vi "Close Item Reference.vi"(8 "error in (no error)":errorcluster, 11 "VI in":refnum<class "VI.lvclass">) -> (0 "error out":errorcluster, 3 "VI out":refnum<class "VI.lvclass">)   [LabVIEW 2020, in "VI Properties Editor.lvlib" / "VI.lvclass"]
doc: "Closes the reference contained within the class data of <B>VI in</B>."
uses:
  VI.lvclass
  VI.lvclass/VI.ctl
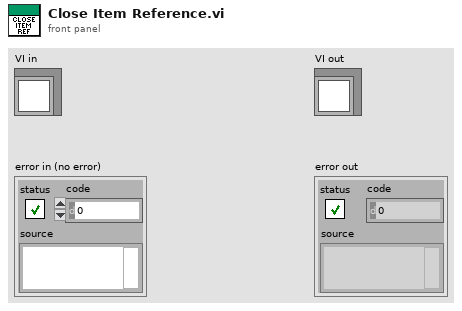
[diagram p1: front panel]
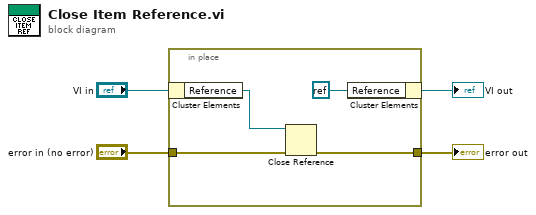
[diagram p0: block diagram]
diagram:
  n1 = in-place {
    in-place-border: "error in (no error)" -> [w8]
    in-place-border: [w5] -> w1
    n2 = in-place-cluster #1("VI in") -> ("Reference"=w6:refnum<vi>)
    n3 = Close Reference(reference=w6, error in (no error)=w8) -> (error out=w5:errorcluster)
    n4 = in-place-cluster #1("Reference"=refnum<k0> refnum) -> (→"VI out":refnum<class "VI.lvclass">)
  }
  "error out" <- w1
